vi "system_config.vi"() -> ()   [LabVIEW 2026]
uses:
  <vilib>/addons/_JKI.lib/Serialization/JSON/JKI JSON Serialization.lvlib
panel:
  in  "Number of Nodes":dbl
  in  "?":T1
  out "Preview":string
  in  "Nodes":T2(array[cluster])
  in  "Clear / Reset":bool
  in  "Generate JSON":bool
  in  "?":bool
  out "Status Message":string
  in  "Save Path":path
  # "Scenario Global Settings"
  # "Actions"
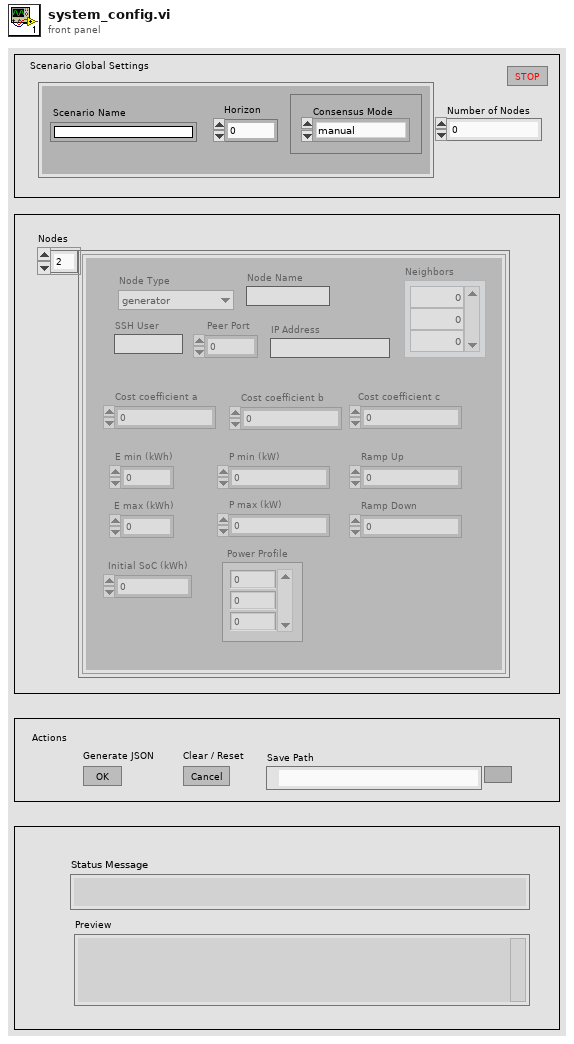
[diagram p1: front panel]
types:
  T1 = cluster{"horizon":i32, "name":string, "consensus":cluster{"mode":enum16{"manual", "auto"}}}
  T2 = cluster{"name":string, "ip":string, "peer_port":dbl, "a":dbl, "b":dbl, "p_min":dbl, "p_max":dbl, "ramp_up":dbl, "ramp_down":dbl, "e_min":dbl, "e_max":dbl, "e_init":dbl, "profile":dbl[], "type":enum16{"generator", "load", "battery"}, "ssh_user":string, "c":dbl, "neighbors":dbl[]}[]
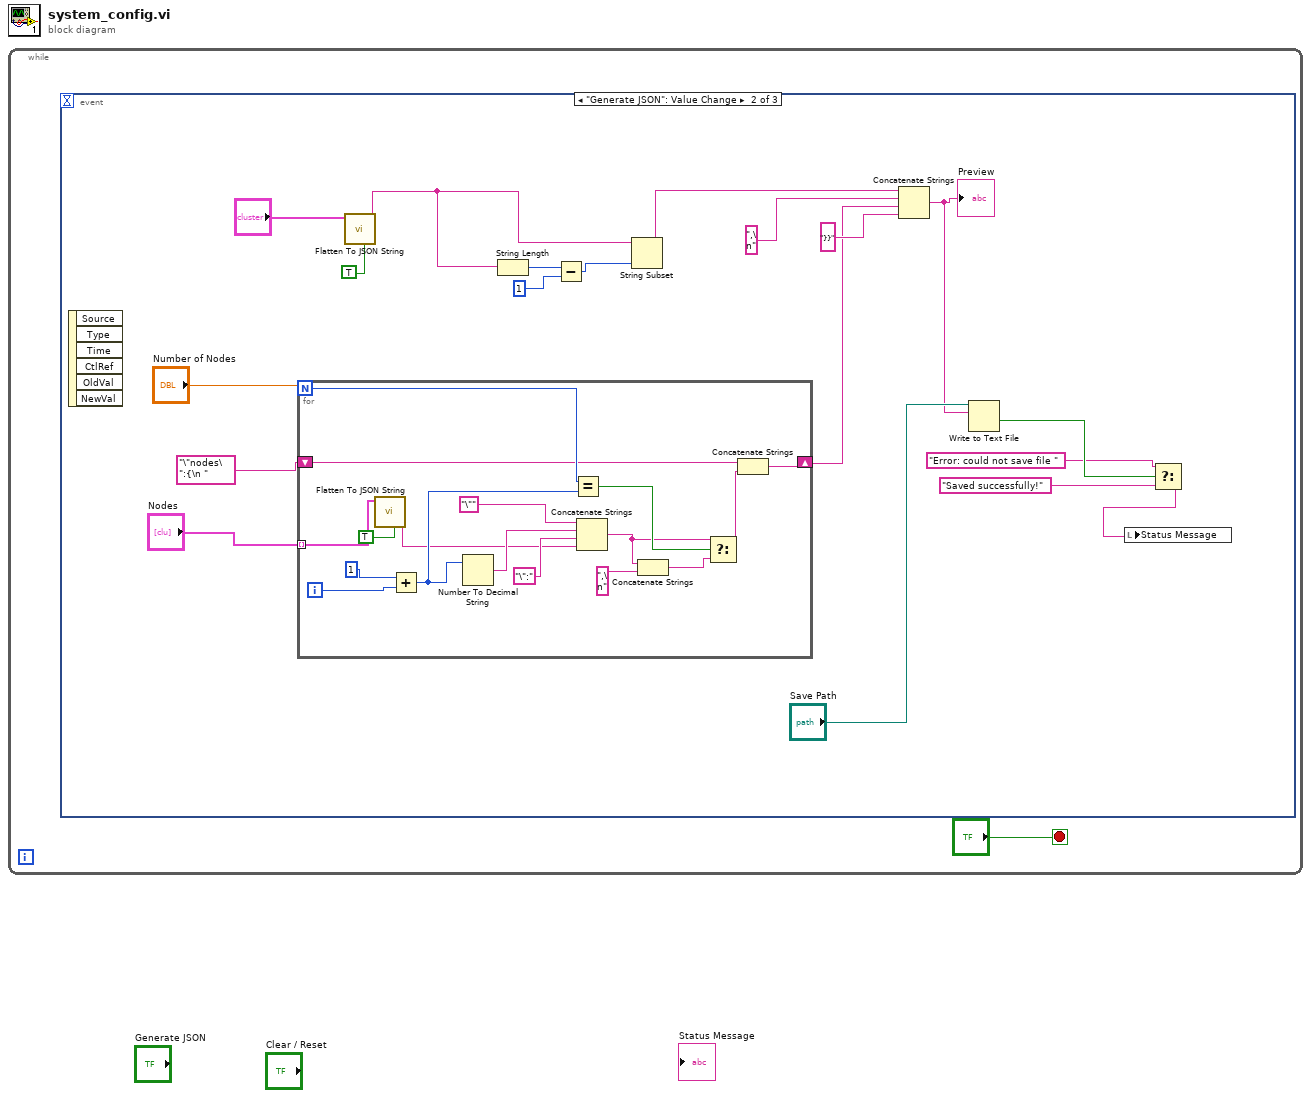
[diagram p0: block diagram]
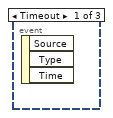
[diagram p2: hidden frame]
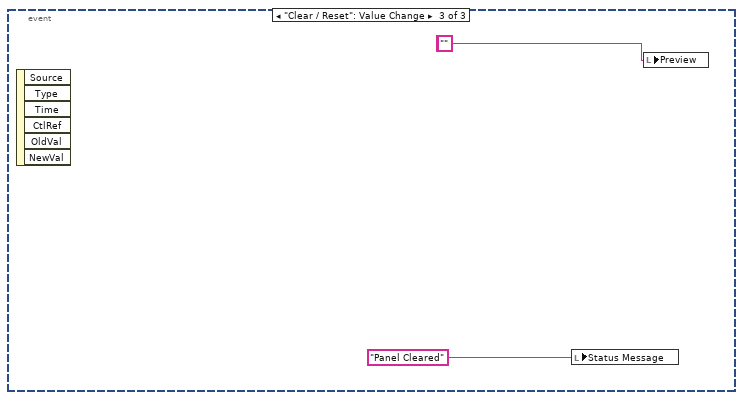
[diagram p3: hidden frame]
diagram:
  n1 = while {
    stop <- "?" stop-if-true
    n2 = event shown="[1] \"Generate JSON\": Value Change" {
      selector: _ -> [_ _ _]
      dyn-events: _ -> [_ _ _]
      timeout: _ -> [_ _ _]
      event Timeout {
        n3 = event-data() -> ()  [unwired: 1 in, 3 out]
      }
      event "Generate JSON": Value Change {
        n4 = event-data() -> ()  [unwired: 1 in, 6 out]
        n5 = for {
          N: "Number of Nodes" -> [w33]
          tunnel: "Nodes" -> [w25] mode=indexing
          shift-right: [w26] -> w11
          shift-left: "\"nodes\":{\n " -> [w28]
          i -> [w37]
          n6 = call <vilib>:"Flatten To JSON String.vi"("Enums As String (F)"=TRUE, "Variant"=w25) -> ("JSON String"=w22:string)  [unwired: 8 in, 1 out]
          n7 = Add(x=1, y=w37) -> (x+y=w34:i32)
          n8 = Number To Decimal String(number=w34) -> (decimal integer string=w24:string)  [unwired: 1 in]
          n9 = Equal?(x=w33, y=w34) -> (x = y?=w31:bool)
          n10 = Concatenate Strings("\"", w24, "\":", w22) -> (w30:string)
          n11 = Concatenate Strings(w30, ",\n") -> (w29:string)
          n12 = Select(t=w30, s=w31, f=w29) -> (s? t:f=w27:string)
          n13 = Concatenate Strings(w28, w27) -> (w26:string)
        }
        n14 = call <vilib>:"Flatten To JSON String.vi"("Enums As String (F)"=TRUE, "Variant"="?") -> ("JSON String"=w15:string)  [unwired: 8 in, 1 out]
        n15 = String Length(string=w15) -> (length=w14:i32)
        n16 = Subtract(x=w14, y=1) -> (x-y=w12:i32)
        n17 = String Subset(string=w15, length (rest)=w12) -> (substring=w16:string)  [unwired: 1 in]
        n18 = Concatenate Strings(w16, ",\n", w11, "}}") -> (w8:string)
        "Preview" <- w8
        n19 = Write to Text File(file (use dialog)="Save Path", text=w8) -> (cancelled=w7:bool)  [unwired: 2 in, 2 out]
        n20 = Select(t="Error: could not save file ", s=w7, f="Saved successfully!") -> (s? t:f=w4:string)
        n21 = local write "Status Message"(w4) -> ()
      }
      event "Clear / Reset": Value Change {
        (unwired) ""
        n22 = event-data() -> ()  [unwired: 1 in, 6 out]
        n23 = local write "Status Message"("Panel Cleared") -> ()
        n24 = local write "Preview"("") -> ()
      }
    }
  }
